vi "Read Publisher Info.vi"(8 "error in (no error)":errorcluster, 9 "timeout_ms":u32=5000, 10 "Topic":string, 11 "Name":string) -> (0 "error out":errorcluster, 3 "Publisher Info":T1)   [LabVIEW 2021, in "Iceoryx.lvlib"]
uses:
  Iceoryx.lvlib
  typedef/Publisher Info.ctl
  SubVIs/Convert Error Core.vi
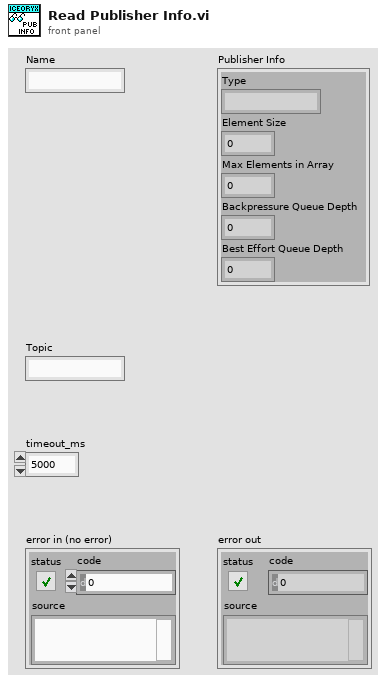
[diagram p1: front panel]
types:
  T1 = typedef "Iceoryx.lvlib/Publisher Info.ctl" = cluster{"Type":string, "Element Size":u32, "Max Elements in Array":u32, "Backpressure Queue Depth":u32, "Best Effort Queue Depth":u32}
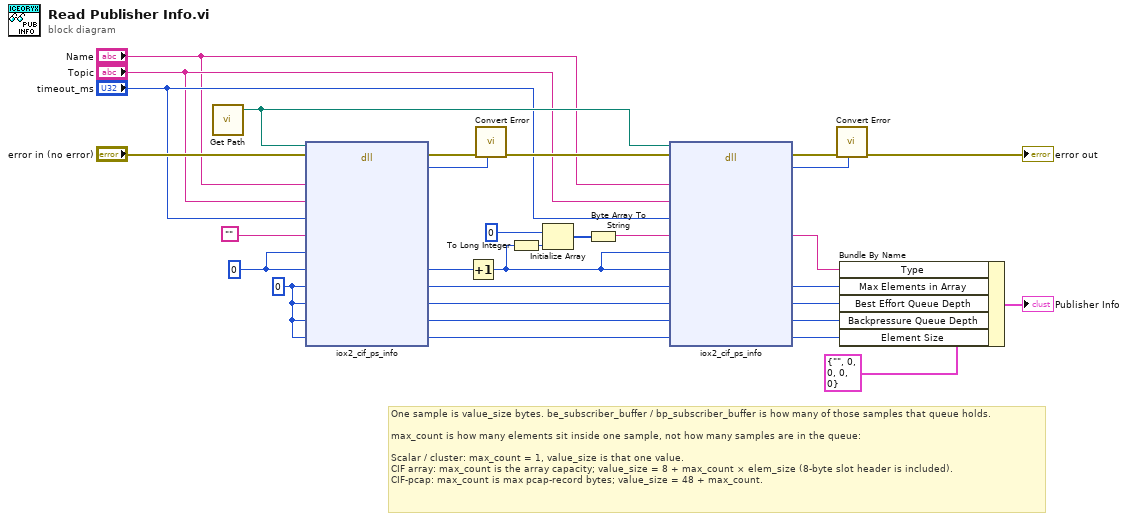
[diagram p0: block diagram]
diagram:
  w15 = u32 0 ("max_count")
  w28 = u32 0 ("actual")
  # "One sample is value_size bytes. be_subscriber_buffer / bp_subscriber_buffer is how many of those samples that queue holds.\n\nmax_count is how many elements sit inside one sample, not how many samples are in the queue:\n\nScalar / cluster: max_count = 1, value_size is that one value.\nCIF array: max_count is the array capacity; value_size = 8 + max_count × elem_size (8-byte slot header is included).\nCIF-pcap: max_count is max pcap-record bytes; value_size = 48 + max_count."
  n1 = call "Get Path.vi"() -> ("libiox2_cif path"=w20:path)  [unwired: 4 in]
  n2 = dll-call lib="D:/dev/iceoryx2_lvwrapper/dist/iox2_cif.dll" fn="iox2_cif_ps_info"(path in=w20, error in="error in (no error)", "name"="Name", "topic"="Topic", "timeout_ms"="timeout_ms", "type_name"="", "type_cap"=w28, "type_len"=w28, "max_count"=w15, "be_subscriber_buffer"=w15, "bp_subscriber_buffer"=w15, "value_size"=w15) -> (error out=w30:errorcluster, "return type"=w29:i32, "type_len"=w25:u32, "max_count"=w11:u32, "be_subscriber_buffer"=w12:u32, "bp_subscriber_buffer"=w13:u32, "value_size"=w14:u32)  [unwired: 6 in, 1 out]
  n3 = Increment(x=w25) -> (x+1=w10:u32)
  n4 = call "Convert Error.vi"("return type"=w29, "error in (no error)"=w30) -> ("error out"=w21:errorcluster)  [unwired: 9 in]
  n5 = To Long Integer(number=w10) -> (32bit integer=w23:i32)
  n6 = Initialize Array(u8 0 ("actual"), w23) -> (w22:u8[])
  n7 = Byte Array To String(unsigned byte array=w22) -> (string=w16:string)
  n8 = dll-call lib="D:/dev/iceoryx2_lvwrapper/dist/iox2_cif.dll" fn="iox2_cif_ps_info"(path in=w20, error in=w21, "name"="Name", "topic"="Topic", "timeout_ms"="timeout_ms", "type_name"=w16, "type_cap"=w10, "type_len"=w10, "max_count"=w11, "be_subscriber_buffer"=w12, "bp_subscriber_buffer"=w13, "value_size"=w14) -> (error out=w19:errorcluster, "return type"=w18:i32, "type_name"=w6:string, "max_count"=w7:u32, "be_subscriber_buffer"=w3:u32, "bp_subscriber_buffer"=w4:u32, "value_size"=w5:u32)  [unwired: 6 in, 1 out]
  n9 = call "Convert Error.vi"("return type"=w18, "error in (no error)"=w19) -> ("error out"=→"error out":errorcluster)  [unwired: 9 in]
  n10 = Bundle By Name(cluster=T1 {"Type"="", "Element Size"=0, "Max Elements in Array"=0, "Backpressure Queue Depth"=0, "Best Effort Queue Depth"=0} ("Publisher Info"), "Type"=w6, "Max Elements in Array"=w7, "Best Effort Queue Depth"=w3, "Backpressure Queue Depth"=w4, "Element Size"=w5) -> (→"Publisher Info":T1)
